vi "TCP Receive.vi"() -> ()   [LabVIEW 2018]
doc: "Demonstrates how to set up a basic TCP connection, send data to the specified port once a connection has been established, and terminate the connection once the data has been sent. This VI is designed to stop if the TCP connection is terminated. The data sent in this example is an array of random numbers."
panel:
  out "double precision float":dbl[](array[numeric])
  in  "Stop":bool
  # "Overview: Demonstrates the use of the TCP functions to initialize a TCP server that can send data to a client VI.\nInstructions:\n1. Run the VI.\n2. Open Simple TCP - Client.vi and follow the instructions on its front panel. Note that if you wait longer than 30 seconds to do this after running this VI, it will time out.\n3. Click Stop to stop the VI. Note that if you stop the client VI, this VI will stop automatically."
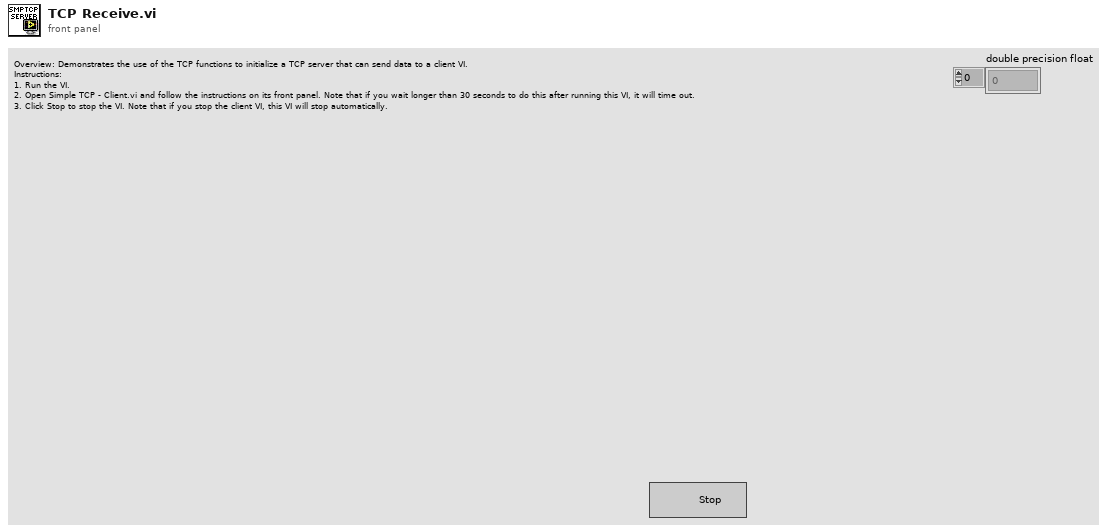
[diagram p1: front panel]
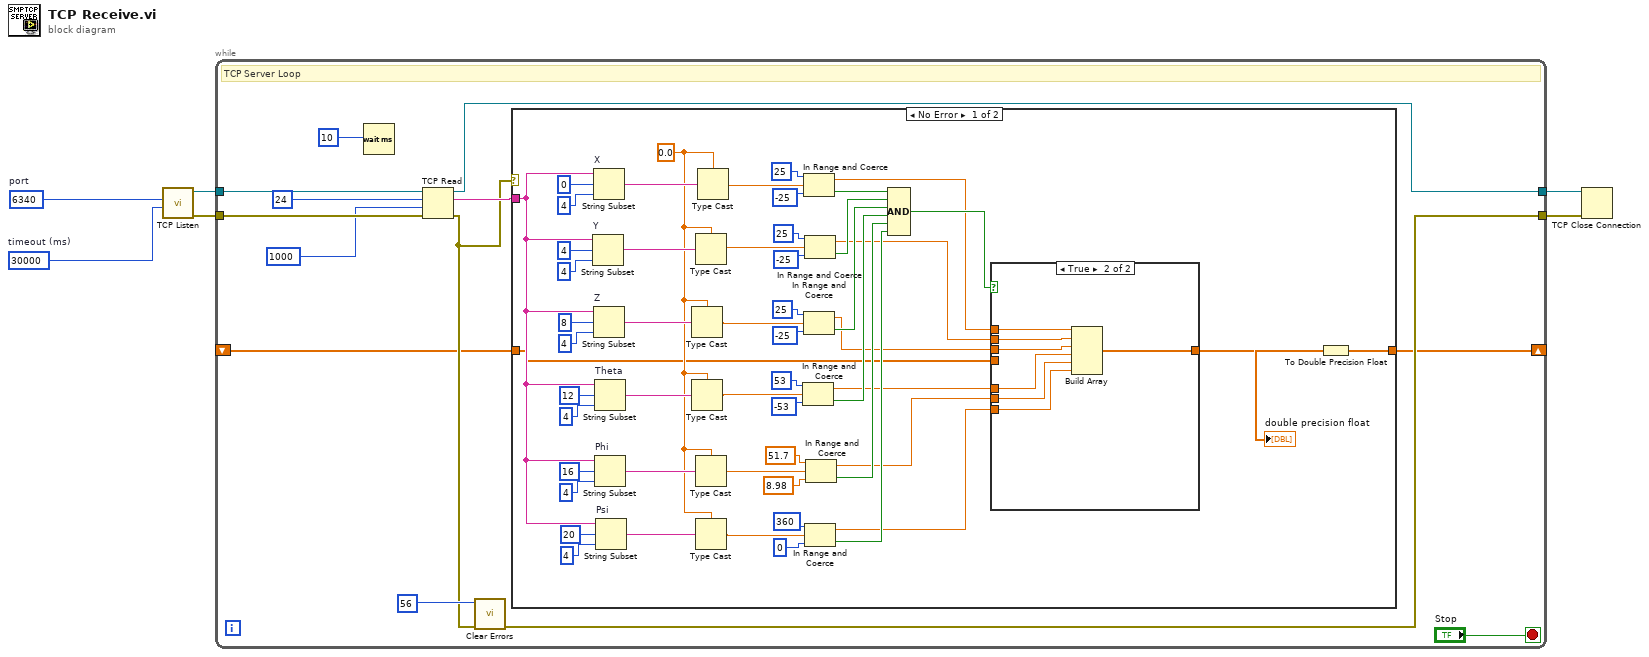
[diagram p0: block diagram]
diagram:
  w2 = u16 6340  # port
  w3 = 30000  # timeout (ms)
  n1 = call <vilib>:"TCP Listen.vi"("timeout ms (wait forever: -1)"=w3, "port"=w2) -> ("error out"=w4:errorcluster, "connection ID"=w5:refnum<k5>)  [unwired: 5 in, 3 out]
  n2 = while {
    tunnel: [w14] -> w6
    tunnel: w5 -> [w17]
    tunnel: w4 -> [w18]
    tunnel: [w11] -> w1
    shift-right: [w8] -> _
    shift-left: _ -> [w7]
    stop <- "Stop" stop-if-true
    # "TCP Server Loop"
    n3 = Wait (ms)(milliseconds to wait=10) -> ()  [unwired: 1 out]
    n4 = TCP Read(connection ID=w17, bytes to read=24, error in (no error)=w18, 9:1000 ("timeout ms (25000)")) -> (connection ID out=w11:refnum<k5>, data out=w12:string, error out=w10:errorcluster)  [unwired: 1 out]
    n5 = call <vilib>:"Clear Errors.vi"("error in (no error)"=w10, "specific error code to clear (0: all)"=56) -> ("error out"=w14:errorcluster)  [unwired: 4 in, 1 out]
    n6 = case shown="No Error" w10 {
      tunnel: w12 -> [w60 _]
      tunnel: [w53 w82] -> w8
      tunnel: w7 -> [w20 w82]
      frame No Error {
        w54 = sgl 0.0 ("x")
        n7 = String Subset "Y"(string=w60, offset (0)=4, length (rest)=4) -> (substring=w59:string)
        n8 = String Subset "X"(string=w60, offset (0)=0, length (rest)=4) -> (substring=w61:string)
        n9 = String Subset "Z"(string=w60, offset (0)=8, length (rest)=4) -> (substring=w58:string)
        n10 = String Subset "Theta"(string=w60, offset (0)=12, length (rest)=4) -> (substring=w57:string)
        n11 = String Subset "Phi"(string=w60, offset (0)=16, length (rest)=4) -> (substring=w56:string)
        n12 = String Subset "Psi"(string=w60, offset (0)=20, length (rest)=4) -> (substring=w55:string)
        n13 = Type Cast(type=w54, x=w58) -> (*(type *) &x=w38:sgl)
        n14 = Type Cast(type=w54, x=w57) -> (*(type *) &x=w37:sgl)
        n15 = Type Cast(type=w54, x=w59) -> (*(type *) &x=w39:sgl)
        n16 = Type Cast(type=w54, x=w56) -> (*(type *) &x=w36:sgl)
        n17 = Type Cast(type=w54, x=w55) -> (*(type *) &x=w35:sgl)
        n18 = Type Cast(type=w54, x=w61) -> (*(type *) &x=w52:sgl)
        n19 = In Range and Coerce(upper limit=53, x=w37, lower limit=-53) -> (coerced(x)=w23:sgl, In Range?=w30:bool)
        n20 = In Range and Coerce(upper limit=25, x=w52, lower limit=-25) -> (coerced(x)=w26:sgl, In Range?=w33:bool)
        n21 = In Range and Coerce(upper limit=25, x=w38, lower limit=-25) -> (coerced(x)=w24:sgl, In Range?=w31:bool)
        n22 = In Range and Coerce(upper limit=25, x=w39, lower limit=-25) -> (coerced(x)=w25:sgl, In Range?=w32:bool)
        n23 = In Range and Coerce(upper limit=360, x=w35, lower limit=0) -> (coerced(x)=w21:sgl, In Range?=w28:bool)
        n24 = In Range and Coerce(upper limit=51.7, x=w36, lower limit=8.98) -> (coerced(x)=w22:dbl, In Range?=w29:bool)
        n25 = Compound Arithmetic op=AND(w33, w32, w31, w30, w29, w28) -> (w34:bool)
        n26 = case shown="True" w34 {
          tunnel: [w74 w81] -> w27
          tunnel: w26 -> [_ w80]
          tunnel: w25 -> [_ w79]
          tunnel: w24 -> [_ w78]
          tunnel: w23 -> [_ w77]
          tunnel: w22 -> [_ w76]
          tunnel: w21 -> [_ w75]
          tunnel: w20 -> [w74 _]
          frame False {
          }
          frame True {
            n27 = Build Array(w80, w79, w78, w77, w76, w75) -> (w81:dbl[])
          }
        }
        n28 = To Double Precision Float(number=w27) -> (double precision float=w53:dbl[])
        "double precision float" <- w53
      }
      frame Error {
      }
    }
  }
  n29 = TCP Close Connection(connection ID=w1, error in (no error)=w6) -> ()  [unwired: 3 out]
